vi "Get Queue.vi"(8 "error in (no error)":errorcluster, 10 "ID":string, 11 "uService List in":refnum<class "uService List.lvclass">) -> (0 "error out":errorcluster, 2 "uService Queue":refnum<class "Message Enqueuer.lvclass">, 3 "uService List out":refnum<class "uService List.lvclass">)   [LabVIEW 2020, in "TALOS.lvlib" / "Classes.lvlib" / "uService List.lvclass"]
uses:
  uService List.lvclass
  TALOS.lvlib
  builds/Actor Framework PPL/Actor Framework.lvlibp/1abvi3w/vi.lib/ActorFramework/Message Enqueuer/Message Enqueuer.lvclass
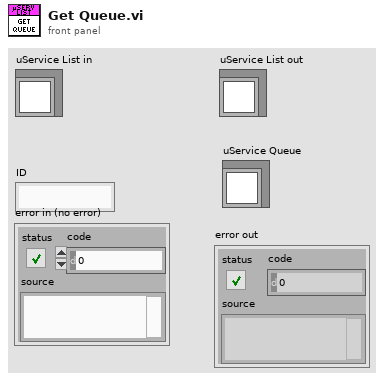
[diagram p1: front panel]
types:
  T1 = typedef "TALOS.lvlib/Classes.lvlib/uService List.lvclass/uService Properties.ctl" = cluster{"uService Queue":refnum<class "Message Enqueuer.lvclass">, "Last Pat":timestamp, "Online":bool, "Vi Ref":refnum<vi>, "Class name":string, "GUI":bool, "FP Items Refs Map":map{string, refnum<vi>}}
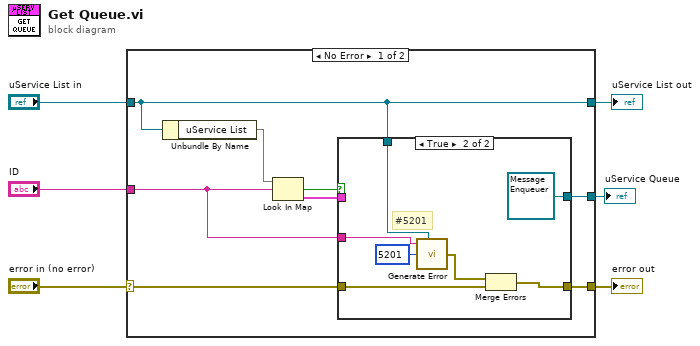
[diagram p0: block diagram]
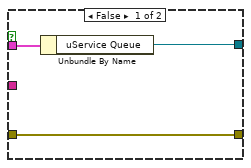
[diagram p2: hidden frame]
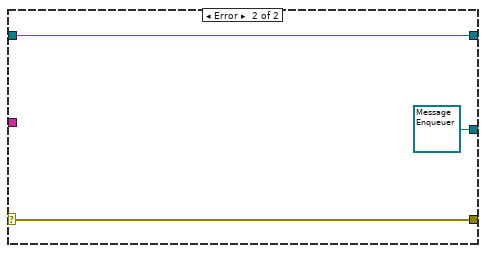
[diagram p3: hidden frame]
diagram:
  n1 = case shown="No Error" "error in (no error)" {
    selector: "error in (no error)" -> [w13 w27]
    tunnel: "uService List in" -> [w8 w26]
    tunnel: [w11 w27] -> w4
    tunnel: [w8 w26] -> w3
    tunnel: "ID" -> [w7 _]
    tunnel: [w9 refnum<class "Message Enqueuer.lvclass"> refnum ("uService Queue")] -> w1
    frame No Error {
      n2 = Unbundle By Name(w8) -> ("uService List"=w14:map{string, T1})
      n3 = Look In Map(map=w14, key=w7) -> (key not found?=w12:bool, value=w10:T1)  [unwired: 1 in]
      n4 = case shown="True" w12 {
        tunnel: w13 -> [w17 w22]
        tunnel: [w17 w21] -> w11
        tunnel: w10 -> [w16 _]
        tunnel: [w15 refnum<class "Message Enqueuer.lvclass"> refnum ("uService Queue")] -> w9
        tunnel: w8 -> [_ w19]
        tunnel: w7 -> [_ w18]
        frame False {
          n5 = Unbundle By Name(w16) -> ("uService Queue"=w15:refnum<class "Message Enqueuer.lvclass">)
        }
        frame True {
          # "#5201"
          n6 = call "Generate Error.vi"("Optional String"=w18, "Class"=w19, "Error Code"=5201) -> ("error out"=w23:errorcluster)  [unwired: 4 in]
          n7 = Merge Errors(w23, w22) -> (w21:errorcluster)
        }
      }
    }
    frame Error {
    }
  }
  "error out" <- w4
  "uService List out" <- w3
  "uService Queue" <- w1
